vi "Call Commands.vi"(10 "Iterations":i32, 11 "Commands":cluster{"Time (s)":dbl, T1, bool}[](array[cluster])) -> ()   [LabVIEW 2023]
uses:
  bordeaux-main/Bordeaux/Types/Single Cmd Info.ctl
  <vilib>/picture/picture.llb/imagedata.ctl
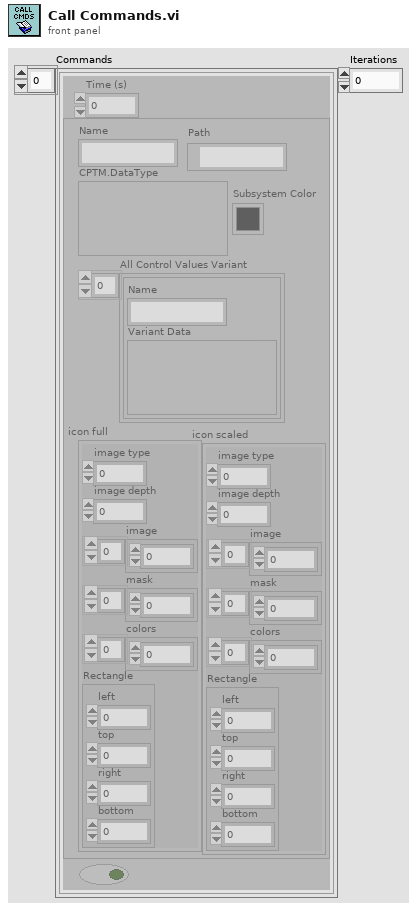
[diagram p1: front panel]
types:
  T1 = typedef "Single Cmd Info.ctl" = cluster{"Name":string, "CPTM.DataType":variant, "All Control Values Variant":cluster{"Name":string, "Variant Data":variant}[], "icon full":T2, "icon scaled":T2, "Path":path, "Subsystem Color":u32}
  T2 = typedef "imagedata.ctl" = cluster{"image type":i32, "image depth":i32, "image":u8[], "mask":u8[], "colors":u32[], "Rectangle":cluster{"left":i16, "top":i16, "right":i16, "bottom":i16}}
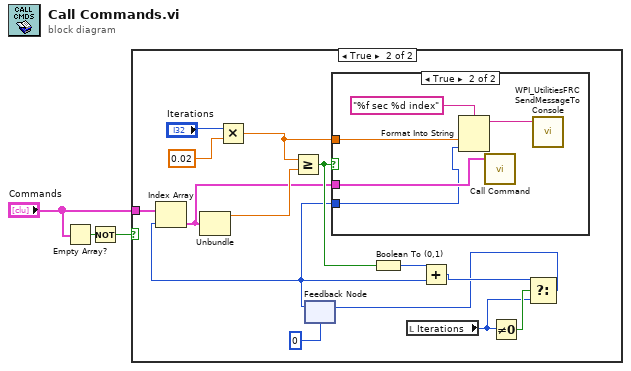
[diagram p0: block diagram]
diagram:
  n1 = Empty Array?(array="Commands") -> (empty?=w2:bool)
  n2 = Not(x=w2) -> (.not. x?=w1:bool)
  n3 = case shown="True" w1 {
    tunnel: "Commands" -> [_ w10]
    frame False {
    }
    frame True {
      n4 = Multiply(x="Iterations", y=0.02) -> (x*y=w5:dbl)
      n5 = feedback #1(i16 0) -> (w4:i32)
      n6 = Index Array(array=w10, index=w4) -> (element=w11:cluster{"Time (s)":dbl, T1, bool})
      n7 = Unbundle(w11) -> ("Time (s)"=w15:dbl)  [unwired: 2 out]
      n8 = Greater Or Equal?(x=w5, y=w15) -> (x >= y?=w14:bool)
      n9 = case shown="True" w14 {
        tunnel: w11 -> [_ w22]
        tunnel: w5 -> [_ w21]
        tunnel: w4 -> [_ w20]
        frame False {
        }
        frame True {
          n10 = Format Into String(format string="%f sec %d index", w21, w20) -> (resulting string=w19:string)  [unwired: 2 in, 1 out]
          n11 = call "Call Command.vi"("Command"=w22) -> ()  [unwired: 11 in]
          n12 = call <vilib>:"WPI_UtilitiesFRC SendMessageToConsole.vi"("Message"=w19) -> ()  [unwired: 14 in, 1 out]
        }
      }
      n13 = Boolean To (0,1)(Boolean=w14) -> (0, 1=w13:i16)
      n14 = local read "Iterations"() -> (w7:i32)
      n15 = Add(x=w13, y=w4) -> (x+y=w9:i32)
      n16 = Not Equal To 0?(x=w7) -> (x != 0?=w8:bool)
      n17 = Select(t=w9, s=w8, f=w7) -> (s? t:f=w6:i32)
      n18 = feedback-in #1(w6) -> ()
    }
  }
